vi "Test MQTT-3.1.0-1.vi"(8 "error in (no error)":errorcluster, 11 "Connection Config":refnum<class "Connection.lvclass">) -> (0 "error out":errorcluster, 3 "Connection Config dup":refnum<class "Connection.lvclass">)   [LabVIEW 2013]
uses:
  <vilib>/LabVIEW Open Source Project/MQTT Control Packets/Control Packets/ControlPacket/ControlPacket.lvclass
  <vilib>/addons/_JKI Toolkits/Caraya/classes/Test/Test.lvclass
  <vilib>/addons/_JKI Toolkits/Caraya/classes/Assert/Assert.lvclass
  <vilib>/LabVIEW Open Source Project/MQTT Control Packets/Control Packets/PUBLISH/PUBLISH.lvclass
  <vilib>/LabVIEW Open Source Project/Connection/Connection/Connection.lvclass
  <vilib>/LabVIEW Open Source Project/MQTT Connection/MQTT_Connection/Connection/Connection.lvclass
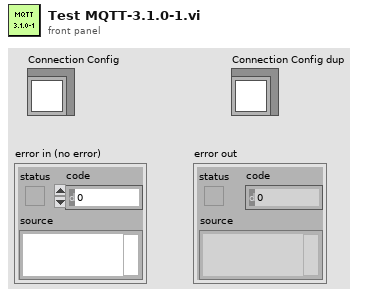
[diagram p1: front panel]
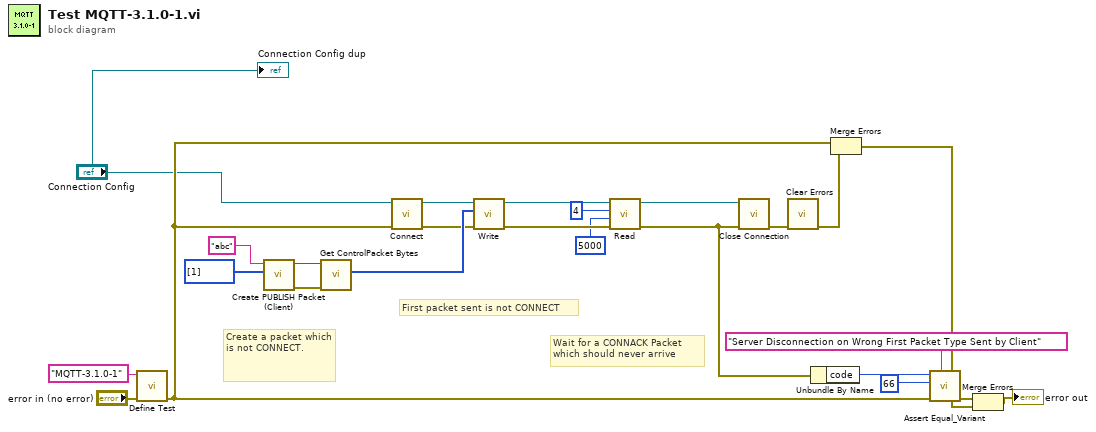
[diagram p0: block diagram]
diagram:
  # "Wait for a CONNACK Packet\nwhich should never arrive"
  # "Create a packet which is not CONNECT."
  # "First packet sent is not CONNECT"
  n1 = call <vilib>:"Define Test.vi"("error in (no error)"="error in (no error)", "Label (VI Title)"="MQTT-3.1.0-1") -> ("error out"=w4:errorcluster)  [unwired: 9 in]
  n2 = call <vilib>:"Create PUBLISH Packet (Client).vi"("Payload"=u8[] [1], "Topic Name"="abc") -> ("error out"=w9:errorcluster, "PUBLISH"=w10:refnum<class "PUBLISH.lvclass">)  [unwired: 6 in, 2 out]
  n3 = call <vilib>:"Get ControlPacket Bytes.vi"("error in (no error)"=w9, "ControlPacket"=w10) -> ("Bytes Stream"=w11:u8[])  [unwired: 6 in, 3 out]
  n4 = call <vilib>:"Connect.vi"("error in (no error)"=w4, "Connection in"="Connection Config") -> ("error out"=w5:errorcluster, "Connection out"=w6:refnum<class "Connection.lvclass">)  [unwired: 8 in]
  n5 = call <vilib>:"Write.vi"("error in (no error)"=w5, "Bytes"=w11, "Connection in"=w6) -> ("error out"=w24:errorcluster, "Connection"=w25:refnum<class "Connection.lvclass">)  [unwired: 7 in]
  n6 = call <vilib>:"Read.vi"("error in (no error)"=w24, "timeout (2000 ms)"=5000 ("timeout ms (25000)"), "bytes to read (100)"=4 ("bytes to read"), "TCPConnection in"=w25) -> ("error out"=w13:errorcluster, "TCPConnection out"=w23:refnum<class "Connection.lvclass">)  [unwired: 3 in, 3 out]
  n7 = call <vilib>:"Close Connection.vi"("error in (no error)"=w13, "Connection in"=w23) -> ("error out"=w17:errorcluster)  [unwired: 8 in, 1 out]
  n8 = call <vilib>:"Clear Errors.vi"("error in (no error)"=w17) -> ("error out"=w12:errorcluster)  [unwired: 6 in]
  n9 = Unbundle By Name(w13) -> ("code"=w19:i32)
  n10 = Merge Errors(w4, w12) -> (w3:errorcluster)
  n11 = call <vilib>:"Assert Equal_Variant.vi"("Label"="Server Disconnection on Wrong First Packet Type Sent by Client", "error in (no error)"=w4, "Y"=66 ("code"), "X"=w19) -> ("error out"=w22:errorcluster)  [unwired: 7 in]
  n12 = Merge Errors(w22, w3) -> (→"error out":errorcluster)
  "Connection Config dup" <- "Connection Config"
